vi "cosCurve.vi"(4 "x":dbl format="%#_13g") -> (0 "減速cos曲線":dbl[](array[numeric]), 1 "加速cos曲線":dbl[](array[numeric]), 2 "曲線迴圈數":i32)   [LabVIEW 2019]
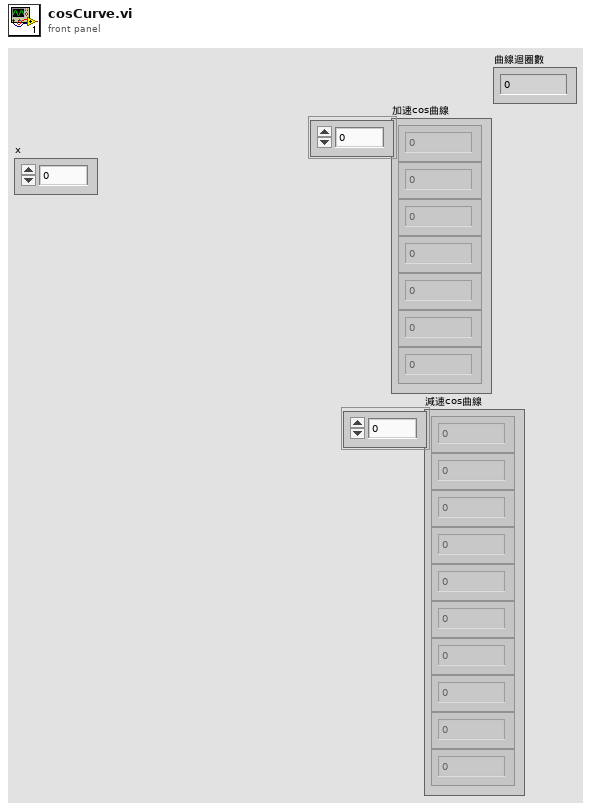
[diagram p1: front panel]
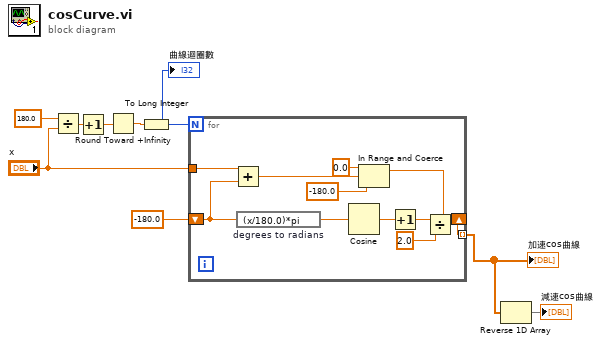
[diagram p0: block diagram]
diagram:
  n1 = Divide(x=180.0, y="x") -> (x/y=w6:dbl)
  n2 = Increment(x=w6) -> (x+1=w5:dbl)
  n3 = Round Toward +Infinity(x=w5) -> (ceil(x): smallest int >= x=w2:dbl)
  n4 = To Long Integer(number=w2) -> (32bit integer=w1:i32)
  "曲線迴圈數" <- w1
  n5 = for {
    N: w1 -> [_]
    shift-right: [w13] -> _
    shift-left: -180.0 -> [w16]
    tunnel: "x" -> [w15]
    tunnel: [w10] -> w4 mode=indexing
    n6 = Add(x=w15, y=w16) -> (x+y=w14:dbl)
    n7 = expression code="(x/180.0)*pi" "degrees to radians"(w16) -> (w20:dbl)
    n8 = Cosine(x=w20) -> (cos(x)=w19:dbl)
    n9 = In Range and Coerce(upper limit=0.0, x=w14, lower limit=-180.0) -> (coerced(x)=w13:dbl)  [unwired: 1 out]
    n10 = Increment(x=w19) -> (x+1=w18:dbl)
    n11 = Divide(x=w18, y=2.0) -> (x/y=w10:dbl)
  }
  "加速cos曲線" <- w4
  n12 = Reverse 1D Array(array=w4) -> (reversed array=→"減速cos曲線":dbl[])
